vi "Report Progress.vi"(8 "error in":errorcluster, 9 "message":string, 10 "total":dbl=nan, 11 "progress":dbl) -> (0 "error out":errorcluster, 3 "cancelled?":bool)   [LabVIEW 2020, in "MCP Server.lvlib"]
doc: "Call this from a tool VI to report how far a long tools/call has got, and to learn whether the client has given up.\n\nWhen the client asked for progress (params._meta.progressToken) and accepts Server-Sent Events (Accept: text/event-stream), the tools/call is answered as an SSE stream and every call here sends {\"jsonrpc\":\"2.0\",\"method\":\"notifications/progress\",\"params\":{\"progressToken\":..,\"progress\":..,\"total\":..,\"message\":..}} as one event, before the final result. Otherwise this VI does nothing and cancelled? is FALSE.\n\nprogress must grow: a value that is not greater than the last one sent is dropped (MCP requires strictly increasing progress). total is left out when it is NaN or not greater than 0, message when it is empty.\n\ncancelled? is TRUE once the request is cancelled and stays TRUE for the rest of the request:\n- MCP 2026-07-28 (modern): the client closed the stream. After each event this VI waits up to 1 s for the stream to take it; when it does not, the client is gone.\n- MCP 2025-06-18 and older (legacy): additionally, the client sent notifications/cancelled with the id of this request. That arrives at once while the call is streamed; for a call that is not streamed it cannot arrive while the call runs (Process HTTP Request.vi handles one request at a time), so it has no effect.\nWhen cancelled? is TRUE, stop working and return: the server sends nothing more for this request.\n\nUse Cancel Requested.vi in loops that do not report progress."
uses:
  MCP Server.lvlib
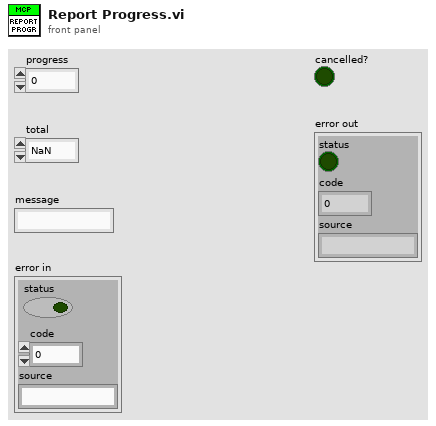
[diagram p1: front panel]
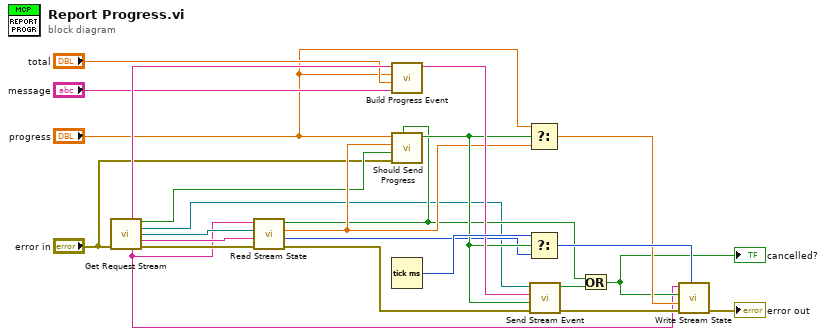
[diagram p0: block diagram]
diagram:
  n1 = call "Get Request Stream.vi"("error in"="error in") -> ("progressToken"=w5:string, "streaming?"=w7:bool, "events"=w8:refnum<queue>, "cancelled"=w9:refnum<queue>, "request id"=w10:string, "stream key"=w6:string, "error out"=w11:errorcluster)  [unwired: 8 in]
  n2 = call "Read Stream State.vi"("error in"=w11, "request id"=w10, "cancelled"=w9, "stream key"=w6) -> ("error out"=w15:errorcluster, "last probe"=w14:u32, "last progress"=w13:dbl, "cancelled?"=w12:bool)  [unwired: 4 in]
  n3 = call "Build Progress Event.vi"("message"="message", "total"="total", "progress"="progress", "progressToken"=w5) -> ("event"=w17:string)  [unwired: 7 in]
  n4 = call "Should Send Progress.vi"("cancelled?"=w12, "error in"="error in", "streaming?"=w7, "last progress"=w13, "progress"="progress") -> ("send?"=w16:bool)  [unwired: 5 in, 1 out]
  n5 = Tick Count (ms)() -> (millisecond timer value=w21:u32)
  n6 = Select(t="progress", s=w16, f=w13) -> (s? t:f=w22:dbl)
  n7 = Select(t=w21, s=w16, f=w14) -> (s? t:f=w23:u32)
  n8 = call "Send Stream Event.vi"("error in"=w15, "send?"=w16, "event"=w17, "events"=w8) -> ("error out"=w19:errorcluster, "client gone?"=w18:bool)  [unwired: 6 in]
  n9 = Or(x=w12, y=w18) -> (x .or. y?=w20:bool)
  "cancelled?" <- w20
  n10 = call "Write Stream State.vi"("last probe"=w23, "error in"=w19, "last progress"=w22, "cancelled?"=w20, "stream key"=w6) -> ("error out"=→"error out":errorcluster)  [unwired: 6 in]
